vi "Process Data.vi"(8 "error in (no error)":errorcluster, 10 "UI Refs":T1, 11 "H1 Hydraulic":refnum<class "H1 Hydraulic.lvclass">) -> (0 "error out":errorcluster, 3 "H1 Hydraulic out":refnum<class "H1 Hydraulic.lvclass">)   [LabVIEW 2025, in "H1 Plotter.lvlib" / "H1 Hydraulic.lvclass"]
uses:
  H1 Hydraulic.lvclass
  H1 Hydraulic.lvclass/H1 Hydraulic.ctl
  Users/Public/Documents/Sandia National Labs/TSS Plugin/Tests/XY Plotter.lvlibp/XY  Plotter/XY Plotter.lvclass
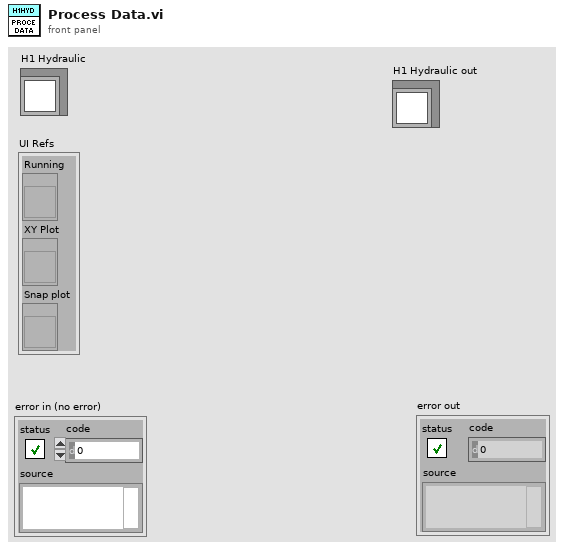
[diagram p1: front panel]
types:
  T1 = cluster{"Running":refnum<vi>, "XY Plot":refnum<vi>, "Snap plot":refnum<vi>}
  T2 = cluster{"Active Plot":u32, "XY Data":cluster{"X":dbl[], "Y":dbl[]}}
  T3 = cluster{"Active Plot":u32, "XY Data":cluster{"X":dbl[], "Y":dbl[]}}[]
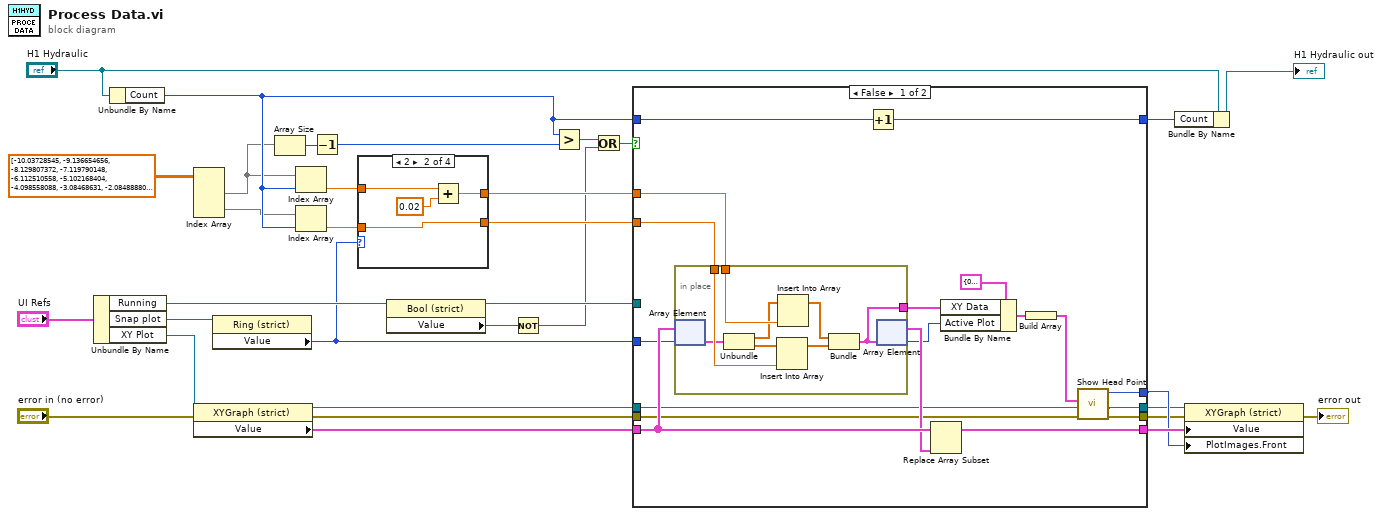
[diagram p0: block diagram]
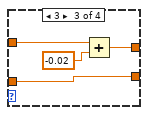
[diagram p3: hidden frame]
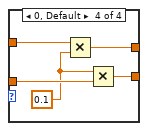
[diagram p4: hidden frame]
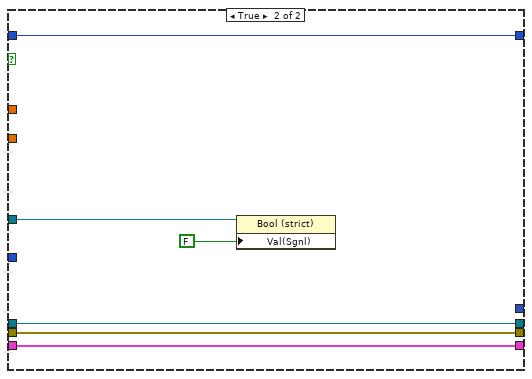
[diagram p5: hidden frame]
diagram:
  n1 = Unbundle By Name("UI Refs") -> ("Running"=w28:refnum<vi>, "Snap plot"=w32:refnum<vi>, "XY Plot"=w31:refnum<vi>)
  n2 = Unbundle By Name("H1 Hydraulic") -> ("Count"=w24:i32)
  n3 = Index Array(array=dbl[][] [[-10.03728545, -9.136654656, -8.129807372, -7.119790148, -6.112510558, -5.102168404, -4.098558088, -3.08468631, -2.084888802, -1.068307366, -0.991141653, -0.965864625, -0.940668483, -0.915472341, -0.892581464, -0.867587538, -0.841975861, -0.819324344, -0.794431724, -0.769619793, -0.745044504, -0.720899886, -0.695622858, -0.670912035, -0.646245995, -0.620843297, -0.597628874, -0.572675392, -0.548611661, -0.523638746, -0.49538835, -0.472618803, -0.445157839, -0.422752281, -0.397273037, -0.373694625, -0.35007577, -0.325122287, -0.301341659, -0.275093993, -0.248811309, -0.224539937, -0.200678422, -0.176008043, -0.150850064, -0.127233489, -0.101794688, -0.078725187, -0.053906532, -0.026593236, -0.002588197, 0.018955821, 0.041414842, 0.065235914, 0.091160034, 0.114819332, 0.139449268, 0.164200534, 0.186908425, 0.21313686, 0.238130785, 0.263731359, 0.288780524, 0.311212123, 0.336852746, 0.360512044, 0.384090455, 0.409084381, 0.436221798, 0.460487744, 0.484367795, 0.509868946, 0.533793295, 0.560503888, 0.583071219, 0.606690073, 0.633139955, 0.656313934, 0.68268293, 0.706544444, 0.730891277, 0.756777913, 0.781607105, 0.808744522, 0.833657561, 0.855132924, 0.880935713, 0.906172298, 0.928524884, 0.954380645, 0.978403932, 1.006269327, 1.762679317, 2.769287671, 3.77798337, 4.789532469, 5.800014341, 6.805830229, 7.820103754, 8.822411019, 9.83253751, 9.338588069, 8.332886059, 7.326452206, 6.3139191, 5.305547783, 4.292674658, 3.287389579, 2.276470281, 1.267937116, 0.994609343, 0.968859326, 0.944027174, 0.918062612, 0.895009962, 0.869479768, 0.844253691, 0.822293009, 0.79715218, 0.770010942, 0.744116218, 0.720185358, 0.69618032, 0.670509513, 0.645232485, 0.620427989, 0.596255716, 0.571423564, 0.547873562, 0.52337699, 0.499151486, 0.474688453, 0.449042306, 0.424493257, 0.399661105, 0.372511396, 0.348823946, 0.323506475, 0.301222247, 0.278129154, 0.252672105, 0.228181747, 0.201676527, 0.176743562, 0.152593323, 0.127482802, 0.10357611, 0.080158583, 0.054518454, 0.029524528, 0.004754521, -0.017915398, -0.042196511, -0.06903566, -0.092573628, -0.118417552, -0.14357256, -0.168162053, -0.193641297, -0.215318877, -0.238492856, -0.266964901, -0.292929464, -0.316750536, -0.341340029, -0.364635338, -0.389184388, -0.412479697, -0.43731185, -0.462718395, -0.487611015, -0.514558448, -0.539673704, -0.563458869, -0.587679836, -0.612431102, -0.63633306, -0.662742499, -0.685956922, -0.711233951, -0.73752206, -0.7602195, -0.786241769, -0.809025718, -0.834897361, -0.859265502, -0.883603063, -0.906186276, -0.931851855, -0.958423068, -0.982163253, -1.007834702, -1.767409317, -2.773253874, -3.783724862, -4.78850728, -5.801097535, -6.808579335, -7.813958107, -8.826374025], [-9.9413773435, -9.939692131249998, -9.93948406575, -9.944341363249999, -9.9439724075, -9.941823004, -9.93566814425, -9.9391603745, -9.936848839750002, -9.937011955250002, -9.940173606250001, -9.941579809499999, -9.94024724575, -9.93958749275, -9.941152237250002, -9.9383567115, -9.937682117, -9.9384371375, -9.9367152815, -9.9355212525, -9.93638239575, -9.93420129275, -9.93747184925, -9.933902716250001, -9.933127498750002, -9.933221316000001, -9.932141076249998, -9.93165956025, -9.931575310500001, -9.9307138355, -9.92853121725, -9.9273084865, -9.926313534250001, -9.925505719250001, -9.925701770499998, -9.92400903925, -9.921302257999999, -9.9192620585, -9.91522659125, -9.91143310775, -9.90308284325, -9.8965172015, -9.89003860975, -9.8779029355, -9.857906684250002, -9.829594956749999, -9.78667253325, -9.709653715999998, -9.579729532750001, -9.337060203, -8.80221734625, -8.096529794999999, -6.650606296000001, -4.43123313875, -1.2280263025000004, 2.0925598750000005, 4.8297741502500005, 6.9043321915, 8.288153131, 9.02631216675, 9.390870275, 9.58738429675, 9.694476303, 9.7595926935, 9.804982938750001, 9.83154606225, 9.85004964625, 9.86688810775, 9.8763347065, 9.88519473275, 9.890961323, 9.8958609185, 9.900022821499999, 9.900893804999999, 9.906576730249999, 9.91019291575, 9.9102057635, 9.9111578735, 9.912169958499998, 9.914168370999999, 9.91388774825, 9.9160095565, 9.91568314875, 9.916328203499999, 9.91780826225, 9.91926072675, 9.918890425, 9.91893765825, 9.92023710075, 9.919306697749999, 9.917936434000001, 9.91628112025, 9.923013185750001, 9.926134823, 9.924495576750001, 9.923771598, 9.922696231249999, 9.921819629000002, 9.9207561425, 9.91863835975, 9.91750932825, 9.91841795925, 9.91262362, 9.916060118750002, 9.918185801749999, 9.91870872125, 9.9168989775, 9.919624163750001, 9.918746137, 9.91810301125, 9.91537127225, 9.915198752, 9.914794091, 9.911406441, 9.909113237749999, 9.911178848250001, 9.911606254, 9.912767936000002, 9.909097670249999, 9.90891240075, 9.91027282325, 9.91031476475, 9.911054807249998, 9.9065752525, 9.90655452275, 9.90498186075, 9.903971855250001, 9.90345735875, 9.901320541750001, 9.901324359750001, 9.897673203499998, 9.90019469525, 9.8970940665, 9.894553169, 9.889803585000001, 9.8860520555, 9.882727375, 9.876984376, 9.86856507725, 9.85815569175, 9.84622852875, 9.83075619575, 9.8083197165, 9.78407483925, 9.74087714575, 9.681881861499999, 9.5918168435, 9.4519164555, 9.178473931500001, 8.72592755875, 7.9803545395, 6.67955623875, 4.791194798749999, 2.1242404125000003, -1.2699715899999995, -4.036155867499999, -6.55895544975, -8.275062827500001, -9.1672003825, -9.5576083975, -9.72258473075, -9.805321267750001, -9.858297709999999, -9.888210627000001, -9.904351233749999, -9.914794396749999, -9.92441091175, -9.93029261825, -9.935031440749999, -9.932615162749999, -9.940193318999999, -9.939432373, -9.94176046775, -9.94158181975, -9.943181933500002, -9.944200279, -9.944239763, -9.944909899499999, -9.945475226500001, -9.94645428125, -9.94445450625, -9.945206936750001, -9.942844433500001, -9.94497052625, -9.94140718675, -9.938964776750002, -9.94183487575, -9.94330821825, -9.943716509000001, -9.94227147275, -9.945753966, -9.942258664999999, -9.9480555705, -9.945226529249998, -9.945823533, -9.946082809, -9.944396053250001, -9.942425435250001, -9.947909416, -9.942300373]] ("appended array")) -> (element #1=w6:dbl[], element #2=w5:dbl[])  [unwired: 4 in]
  n4 = property class="XYGraph (strict)"(reference=w31, error in="error in (no error)") -> (reference out=w13:refnum<vi>, error out=w14:errorcluster, "Value"=w30:cluster{dbl[], dbl[]}[])
  n5 = property class="Ring (strict)"(reference=w32) -> ("Value"=w20:u16)  [unwired: 1 in, 2 out]
  n6 = Array Size(array=w6) -> (size(s)=w4:i32)
  n7 = Index Array(array=w6, index=w24) -> (element=w1:dbl)
  n8 = Index Array(array=w5, index=w24) -> (element=w2:dbl)
  n9 = Decrement(x=w4) -> (x-1=w23:i32)
  n10 = case shown="2" w20 {
    tunnel: [w34 w38 w42 w43] -> w21
    tunnel: w2 -> [w34 w38 w42 w46]
    tunnel: w1 -> [w33 w36 w40 w47]
    tunnel: [w33 w37 w41 w44] -> w22
    frame 1 {
    }
    frame 2 {
      n11 = Add(x=w36, y=0.02 ("Value")) -> (x+y=w37:dbl)
    }
    frame 3 {
      n12 = Add(x=w40, y=-0.02 ("Value")) -> (x+y=w41:dbl)
    }
    frame 0, Default {
      w45 = 0.1 ("Value")
      n13 = Multiply(x=w47, y=w45) -> (x*y=w44:dbl)
      n14 = Multiply(x=w45, y=w46) -> (x*y=w43:dbl)
    }
  }
  n15 = property class="Bool (strict)"(reference=w28) -> (reference out=w19:refnum<vi>, "Value"=w17:bool)  [unwired: 1 in, 1 out]
  n16 = Not(x=w17) -> (.not. x?=w16:bool)
  n17 = Greater?(x=w24, y=w23) -> (0:w18:bool)
  n18 = Or(x=w18, y=w16) -> (x .or. y?=w15:bool)
  n19 = case shown="False" w15 {
    tunnel: w22 -> [w58 _]
    tunnel: w21 -> [w59 _]
    tunnel: [w65 w76] -> w29
    tunnel: w24 -> [w64 w76]
    tunnel: w19 -> [_ w78]
    tunnel: w30 -> [w63 w77]
    tunnel: [w62 w77] -> w25
    tunnel: w20 -> [w60 _]
    tunnel: w14 -> [w53 w75]
    tunnel: w13 -> [w52 w74]
    tunnel: [w50 _] -> w12
    tunnel: [w49 w74] -> w11
    tunnel: [w48 w75] -> w10
    frame False {
      n20 = in-place {
        in-place-border: w58 -> [w73]
        in-place-border: w59 -> [w72]
        in-place-border: [w66] -> w56
        n21 = in-place-array #1(w63, w60) -> (w67:cluster{dbl[], dbl[]})
        n22 = Unbundle(w67) -> (w69:dbl[], w71:dbl[])
        n23 = Insert Into Array(array=w71, new element=w72) -> (w70:dbl[])  [unwired: 1 in]
        n24 = Insert Into Array(array=w69, new element=w73) -> (w68:dbl[])  [unwired: 1 in]
        n25 = Bundle(w68, w70) -> (w66:cluster{dbl[], dbl[]})  [unwired: 1 in]
        n26 = in-place-array #1(w66) -> (w61:cluster{dbl[], dbl[]}[], w54:i32)
      }
      n27 = Increment(x=w64) -> (x+1=w65:i32)
      n28 = Replace Array Subset(array=w63, new element=w61) -> (w62:cluster{dbl[], dbl[]}[])  [unwired: 1 in]
      n29 = Bundle By Name(cluster=T2 {"Active Plot"=0, "XY Data"={"X"=[], "Y"=[]}} ("Dataset"), "XY Data"=w56, "Active Plot"=w54) -> (w55:T2)
      n30 = Build Array(w55) -> (w51:T3)
      n31 = call "Show Head Point.vi"("error in (no error)"=w53, "XY Plot"=w52, "DataSet"=w51) -> ("error out"=w48:errorcluster, "XY Plot out"=w49:refnum<vi>, "picture out"=w50:picture)  [unwired: 6 in]
    }
    frame True {
      n32 = property class="Bool (strict)"(reference=w78, "Val(Sgnl)"=FALSE ("Value (Signaling)")) -> ()  [unwired: 1 in, 2 out]
    }
  }
  n33 = Bundle By Name(cluster="H1 Hydraulic", "Count"=w29) -> (→"H1 Hydraulic out":refnum<class "H1 Hydraulic.lvclass">)
  n34 = property class="XYGraph (strict)"(reference=w11, error in=w10, "Value"=w25, "PlotImages.Front"=w12) -> (error out=→"error out":errorcluster)  [unwired: 1 out]
